vi "Path to Template.vi"(9 "Selector":i32, 10 "Array":path[](array[path]), 11 "Path":path) -> (3 "resolved path":path)   [LabVIEW 2023]
uses:
  <vilib>/Utility/Symbolic Paths/NI_SymbolicPaths.lvlib
  <vilib>/Utility/Symbolic Paths/Symbolic Path ID--enum.ctl
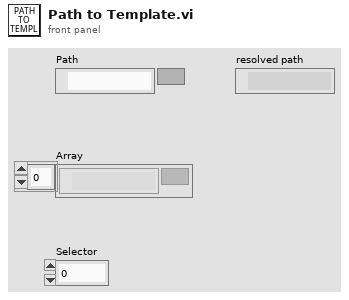
[diagram p1: front panel]
types:
  T1 = typedef "NI_SymbolicPaths.lvlib/Symbolic Path ID--enum.ctl" = enum16{"<invalid>", "<menus>", "<vilib>", "<userlib>", "<instrlib>", "<helpdir>", "<libdir>", "<osdatadir>", "<nishared>", "<instcachedir>", "<resource>", "<extravilib>"}
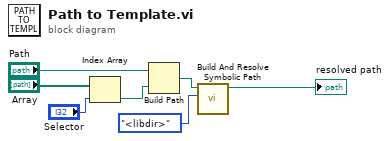
[diagram p0: block diagram]
diagram:
  n1 = Index Array(array="Array", index="Selector") -> (element=w2:path)
  n2 = Build Path(base path="Path", name or relative path=w2) -> (appended path=w6:path)
  n3 = call <vilib>:"Build And Resolve Symbolic Path.vi"("symbolic path id (<vilib>)"=Symbolic_Path_ID--enum."<libdir>" ("symbolic path id"), "relative path"=w6) -> ("resolved path"=→"resolved path":path)  [unwired: 7 in, 2 out]
